vi "Init.vi"(8 "error in (no error)":errorcluster, 11 "Data in":refnum<class "CTI_GPIO_DigitalIn.lvclass">) -> (0 "error out":errorcluster, 3 "Data out":refnum<class "CTI_GPIO_DigitalIn.lvclass">)   [LabVIEW 2021, in "CTI_GPIO_DigitalIn.lvclass"]
doc: "Abstract Data Classes 2.1.1.13\nTim Streeter - TSA\nCopyright (c) 2025, TSA"
uses:
  CTI_GPIO_DigitalIn.lvclass
  <vilib>/CTI/CTI Drivers/CTI/GPIO Direction.ctl
  CTI_GPIO_DigitalIn.lvclass/CTI_GPIO_DigitalIn.ctl
  <vilib>/CTI/CTI Drivers/CTI/Session/Session.lvclass
  <vilib>/CTI/CTI Drivers/CTI/CTI.lvlib
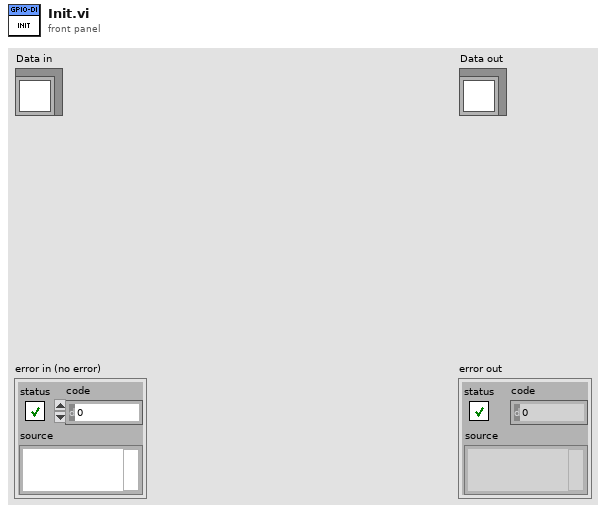
[diagram p1: front panel]
types:
  T1 = typedef "CTI.lvlib/GPIO Direction.ctl" = enum16{"In", "Out"}
  T2 = typedef "CTI.lvlib/GPIO Number.ctl" = i8
  T3 = typedef "CTI.lvlib/GPIO Pull.ctl" = enum16{"None", "Up", "Down", "Both"}
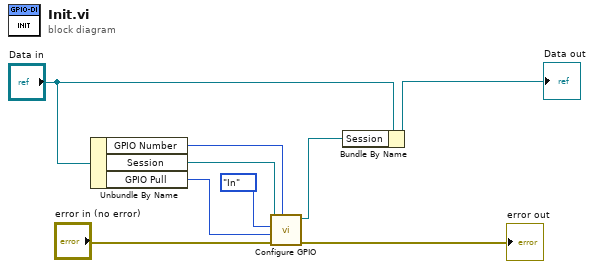
[diagram p0: block diagram]
diagram:
  n1 = Unbundle By Name("Data in") -> ("GPIO Number"=w8:T2, "Session"=w7:refnum<class "Session.lvclass">, "GPIO Pull"=w2:T3)
  n2 = call <vilib>:"Configure GPIO.vi"("GPIO #"=w8, "error in (no error)"="error in (no error)", "GPIO Pull (None)"=w2, "GPIO Direction"=GPIO_Direction."In", "Session in"=w7) -> ("error out"=→"error out":errorcluster, "Session out"=w4:refnum<class "Session.lvclass">)  [unwired: 5 in]
  n3 = Bundle By Name(cluster="Data in", "Session"=w4) -> (→"Data out":refnum<class "CTI_GPIO_DigitalIn.lvclass">)
